vi "Check Sources.vi"(8 "error in (no error)":errorcluster, 11 "EStop Module in":refnum<class "EStop Module.lvclass">) -> (0 "error out":errorcluster, 3 "EStop Module out":refnum<class "EStop Module.lvclass">)   [LabVIEW 2025, in "VolatusControl.lvlib" / "EStop Module.lvclass"]
uses:
  EStop Module.lvclass
  EStop Module.lvclass/EStop Module.ctl
  C:/dev/volatus/mts-volatus-super/libs/lv-volatus/Volatus/Module/Module.lvclass
  C:/dev/volatus/mts-volatus-super/libs/lv-volatus/VolatusControl/EStop Module/EStop Module.lvclass
  Volatus/Module/Module.lvclass
  lv-vecto/Vecto/Vecto.lvlib
  Volatus/VolatusAPI/VolatusAPI.lvclass
  VolatusData/VolatusData.lvlib
  EStop Source/EStop Source.lvclass
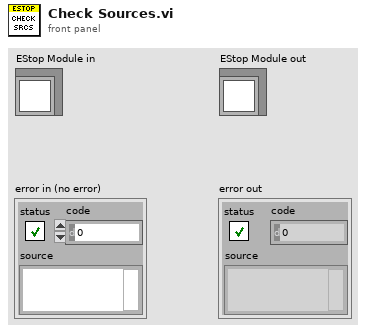
[diagram p1: front panel]
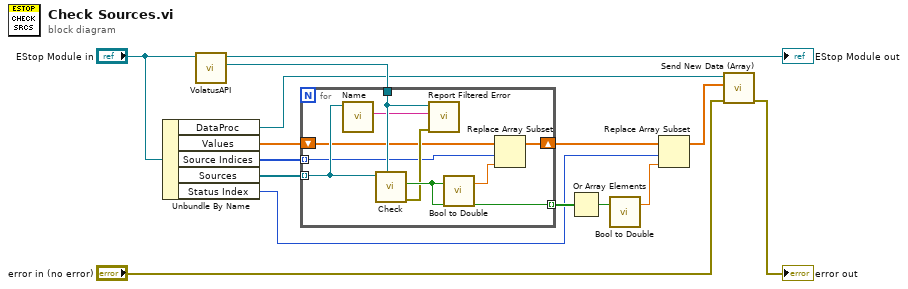
[diagram p0: block diagram]
diagram:
  n1 = Unbundle By Name("EStop Module in") -> ("DataProc"=w4:refnum<class "MessageQ.lvclass">, "Values"=w14:dbl[], "Source Indices"=w13:i32[], "Sources"=w12:refnum<class "EStop Source.lvclass">[], "Status Index"=w5:i32)
  n2 = call "VolatusAPI.vi"("Module in"="EStop Module in") -> ("VolatusAPI"=w10:refnum<class "VolatusAPI.lvclass">, "Module out"=→"EStop Module out":refnum<class "EStop Module.lvclass">)  [unwired: 9 in]
  n3 = for {
    shift-right: [w16] -> w8
    shift-left: w14 -> [w19]
    tunnel: w13 -> [w18] mode=indexing
    tunnel: w12 -> [w21] mode=indexing
    tunnel: w10 -> [w22]
    tunnel: [w24] -> w9 mode=indexing
    n4 = call-dynamic "Name.vi"("EStop Source in"=w21) -> ("Name"=w20:string)  [unwired: 10 in]
    n5 = call-dynamic "Check.vi"("VolatusAPI"=w22, "EStop Source in"=w21) -> ("error out"=w23:errorcluster, "Active"=w24:bool)  [unwired: 7 in, 1 out]
    n6 = call "Report Filtered Error.vi"("error in (no error)"=w23, "Context"=w20, "VolatusAPI in"=w22) -> ()  [unwired: 7 in, 2 out]
    n7 = call "Bool to Double.vi"("Bool"=w24) -> ("Double"=w17:dbl)  [unwired: 2 in]
    n8 = Replace Array Subset(array=w19, new element=w17, index=w18) -> (w16:dbl[])
  }
  n9 = Or Array Elements(Boolean array=w9) -> (logical OR=w7:bool)
  n10 = call "Bool to Double.vi"("Bool"=w7) -> ("Double"=w6:dbl)  [unwired: 2 in]
  n11 = Replace Array Subset(array=w8, new element=w6, index=w5) -> (w3:dbl[])
  n12 = call "Send New Data (Array).vi"("error in (no error)"="error in (no error)", "Data"=w3, "MessageQ"=w4) -> ("error out"=→"error out":errorcluster)  [unwired: 8 in]
